vi "Send Ready for Events Notification.vi"(8 "error in (no error)":errorcluster) -> (0 "error out":errorcluster)   [LabVIEW 2018, in "GLog.lvlib" / "Registry.lvlib"]
uses:
  Registry.lvlib
panel:
  # "Connector Pane"
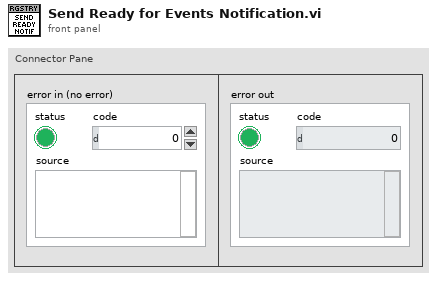
[diagram p1: front panel]
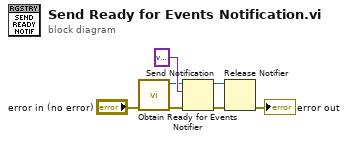
[diagram p0: block diagram]
diagram:
  n1 = call "Obtain Ready for Events Notifier.vi"("error in (no error)"="error in (no error)") -> ("error out"=w3:errorcluster, "notifier"=w2:refnum<notifier>)  [unwired: 9 in]
  n2 = Send Notification(notification=variant, notifier=w2, error in (no error)=w3) -> (notifier out=w6:refnum<notifier>, error out=w5:errorcluster)
  n3 = Release Notifier(notifier=w6, error in (no error)=w5) -> (error out=→"error out":errorcluster)  [unwired: 1 in, 2 out]
